vi "Lint VIs.vi"(8 "error in":errorcluster, 9 "Options":T1={"Force?"=FALSE, "Ignore List"=[], "Only List"=[], "Save(T)?"=TRUE}, 10 "Project Root Folder":path, 11 "IProject Manager in":refnum<class "IProject Manager.lvclass">) -> (0 "error out":errorcluster, 3 "IProject Manager out":refnum<class "IProject Manager.lvclass">)   [LabVIEW 2026, in "IProject Manager.lvclass"]
doc: "Lint project VIs using Blue. The options input parameter is optional."
uses:
  IProject Manager.lvclass
  <vilib>/SAS/blue/blue_core/API/Options--cluster.ctl
  <vilib>/SAS/blue/blue_core/API/API.lvclass
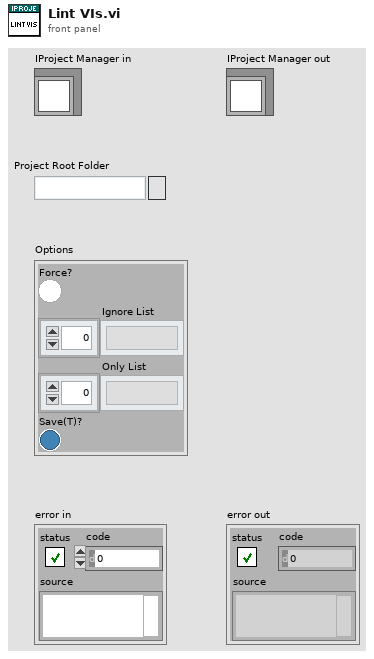
[diagram p1: front panel]
types:
  T1 = typedef "lib_blue_core.lvlib/API.lvclass/Options--cluster.ctl" = cluster{"Force?":bool, "Ignore List":string[], "Only List":string[], "Save(T)?":bool}
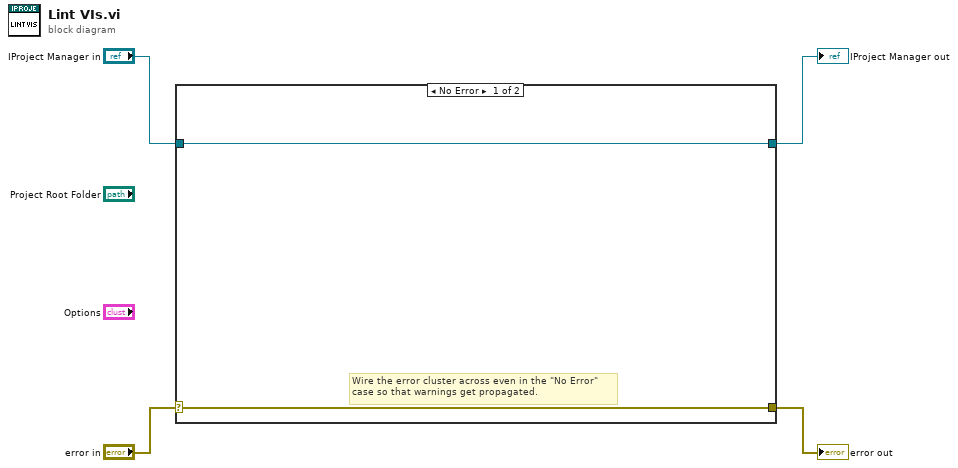
[diagram p0: block diagram]
diagram:
  n1 = case shown="No Error" "error in" {
    selector: "error in" -> [w6 w8]
    tunnel: [w6 w8] -> w3
    tunnel: [w5 w7] -> w1
    tunnel: "IProject Manager in" -> [w5 w7]
    frame No Error {
      # "Wire the error cluster across even in the \"No Error\"\ncase so that warnings get propagated."
    }
    frame Error {
    }
  }
  "error out" <- w3
  "IProject Manager out" <- w1
